vi "W32B Find Control Terminal.vi"(0 "VI reference":refnum<vi>, 5 "label":string, 11 "error in":errorcluster) -> (4 "terminal":refnum<vi>, 15 "error out":errorcluster)   [LabVIEW 2020]
doc: "Returns the block-diagram terminal of the front-panel control or indicator whose label is label, on the VI behind VI reference. A label the panel does not carry leaves terminal invalid and error out set by the property read."
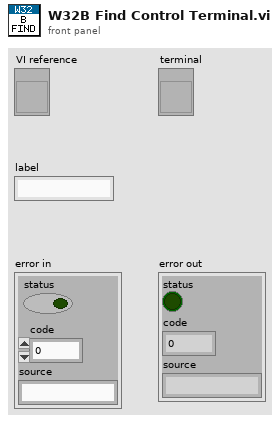
[diagram p1: front panel]
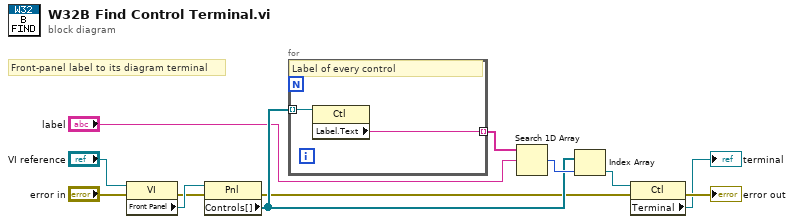
[diagram p0: block diagram]
diagram:
  # "Front-panel label to its diagram terminal"
  n1 = property class="VI"(reference="VI reference", error in="error in") -> (error out=w6:errorcluster, "Front Panel"=w7:refnum<vi>)  [unwired: 1 out]
  n2 = property class="Pnl"(reference=w7, error in=w6) -> (error out=w8:errorcluster, "Controls[]"=w9:refnum<vi>[])  [unwired: 1 out]
  n3 = for {
    tunnel: w9 -> [w13] mode=indexing
    tunnel: [w14] -> w10 mode=indexing
    # "Label of every control"
    n4 = property class="Ctl"(reference=w13) -> ("Label.Text"=w14:string)  [unwired: 1 in, 2 out]
  }
  n5 = Search 1D Array(1D array=w10, element="label") -> (index of element=w11:i32)  [unwired: 1 in]
  n6 = Index Array(array=w9, index=w11) -> (element=w12:refnum<vi>)
  n7 = property class="Ctl"(reference=w12, error in=w8) -> (error out=→"error out":errorcluster, "Terminal"=→"terminal":refnum<vi>)  [unwired: 1 out]
